vi "MecaDrivePoseEst_Kalman_H_Callback.vi"(9 "U":T1, 10 "X":T1, 11 "ExtraPassedData":variant) -> (0 "Error":bool, 3 "Result":T1)   [LabVIEW 2019, in "Trajectory_Library.lvlib"]
doc: "Mecanum Drive Pose Estimator, Kalman Filter H function. \n\nThis function returns row 2 of the X matrix.\n\nInput:\n - ExtraPassedData -- Variant contaiing extra data for the callback For this function the extra data should be empty..\n - X Matrix -- X matrix\n - U Matrix -- U matrix\n\nOutput:\n - Result -- Matrix resulting from calculation\n - Error -- If TRUE an error occured"
uses:
  Trajectory_Library.lvlib
  <vilib>/Analysis/Matrix/Datatypes/RealMatrix.ctl
  <vilib>/Analysis/Matrix/NI_Matrix.lvlib
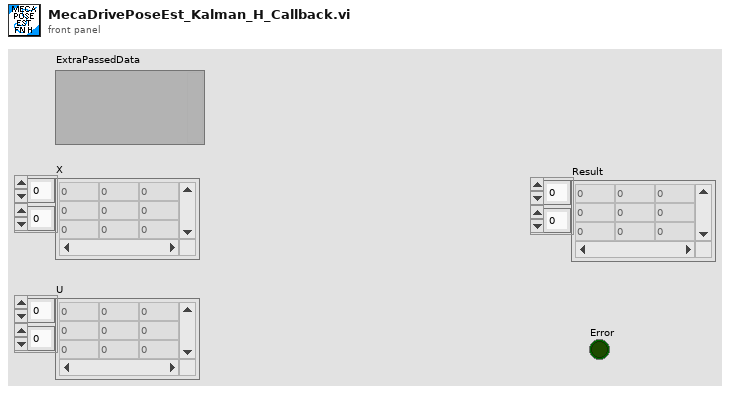
[diagram p1: front panel]
types:
  T1 = typedef "NI_Matrix.lvlib/RealMatrix.ctl" = dbl[][]
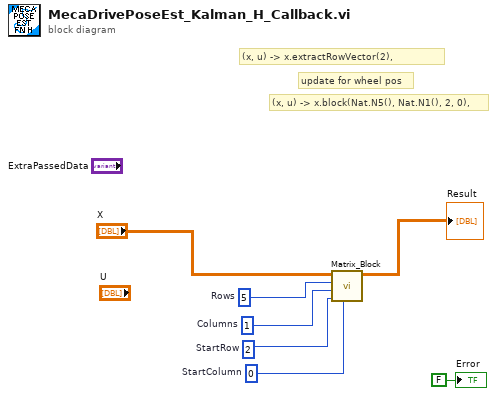
[diagram p0: block diagram]
diagram:
  w3 = 5  # Rows
  w4 = 1  # Columns
  w5 = 2  # StartRow
  w6 = 0  # StartColumn
  # "update for wheel pos"
  # "(x, u) -> x.block(Nat.N5(), Nat.N1(), 2, 0),"
  # "(x, u) -> x.extractRowVector(2),"
  n1 = call "Matrix_Block.vi"("StartColumn"=w6, "StartRow"=w5, "Columns"=w4, "Rows"=w3, "input matrix"="X") -> ("output matrix"=→"Result":T1)  [unwired: 6 in]
  "Error" <- FALSE ("Error")
